vi "RichToFlatcif_can_writer_cansub_InterfaceBlink.vi"(5 "OutputClusterType":T1, 11 "InputCluster":T2) -> (3 "OutputCluster":T1)   [LabVIEW 2021, in "CanWriterCansub_server.lvlib"]
uses:
  CanWriterCansub_server.lvlib
  cif_can_writer_cansub_InterfaceBlink.ctl
  cif_can_writer_cansub_InterfaceBlink_Flat.ctl
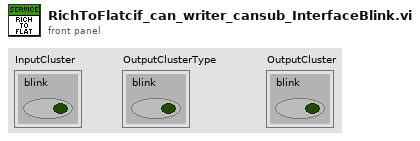
[diagram p1: front panel]
types:
  T1 = typedef "CanWriterCansub_server.lvlib/cif_can_writer_cansub_InterfaceBlink_Flat.ctl" = cluster{"blink":bool}
  T2 = typedef "CanWriterCansub_server.lvlib/cif_can_writer_cansub_InterfaceBlink.ctl" = cluster{"blink":bool}
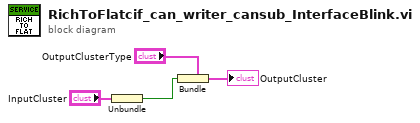
[diagram p0: block diagram]
diagram:
  n1 = Unbundle "Unbundle"("InputCluster") -> ("blink"=w1:bool)
  n2 = Bundle "Bundle"(cluster="OutputClusterType", "blink"=w1) -> (→"OutputCluster":T1)
